vi "LoadNodeUIStandardEvents.vi"(7 "user event out":T1, 8 "error in":errorcluster, 9 "sub panel ref in":refnum<vi>, 10 "main queue":T8, 11 "node":T7) -> (0 "error out":errorcluster)   [LabVIEW 2014, in "NISE_CEF_TreeControl.lvlib"]
doc: "This VI will insert the UI from a node into a subpanel."
uses:
  NISE_CEF_TreeControl.lvlib
  <vilib>/NI/AMC/Message Queue.ctl
  <vilib>/NI/AMC/Message.ctl
  <vilib>/NI/Tools/Keyed Array/KeyedArray.ctl
  Node/NodeRef.ctl
  Node/NISE_CEF_Node.lvclass
  Node/StandardEvents.ctl
  Node/UserEventRef.ctl
  Controls/EventCluster.ctl
  Node/NodeChangeEvent.ctl
  Node/CacheState.ctl
  Node/RefreshUIEvent.ctl
  Node/StopEvent.ctl
  <vilib>/NI/Tools/Keyed Array/Tools_KeyedArray.lvlib
  <vilib>/NI/AMC/AMC.lvlib
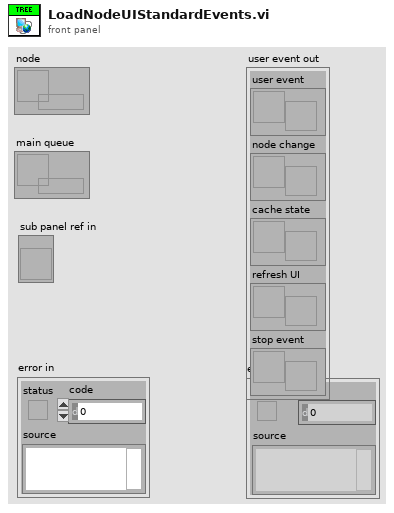
[diagram p1: front panel]
types:
  T1 = typedef "NISE_CEF_Node.lvclass/StandardEvents.ctl" = cluster{"user event":T2, "node change":T3, "cache state":T4, "refresh UI":T5, "stop event":T6}
  T2 = typedef "NISE_CEF_Node.lvclass/UserEventRef.ctl" = refnum<user-event>
  T3 = typedef "NISE_CEF_Node.lvclass/NodeChangeEvent.ctl" = refnum<user-event>
  T4 = typedef "NISE_CEF_Node.lvclass/CacheState.ctl" = refnum<user-event>
  T5 = typedef "NISE_CEF_Node.lvclass/RefreshUIEvent.ctl" = refnum<user-event>
  T6 = typedef "NISE_CEF_Node.lvclass/StopEvent.ctl" = refnum<user-event>
  T7 = typedef "NISE_CEF_Node.lvclass/NodeRef.ctl" = refnum<data-value>
  T8 = typedef "AMC.lvlib/Message Queue.ctl" = refnum<queue>
  T9 = enum32{"Bad", "Idle", "Run top level", "Running"}
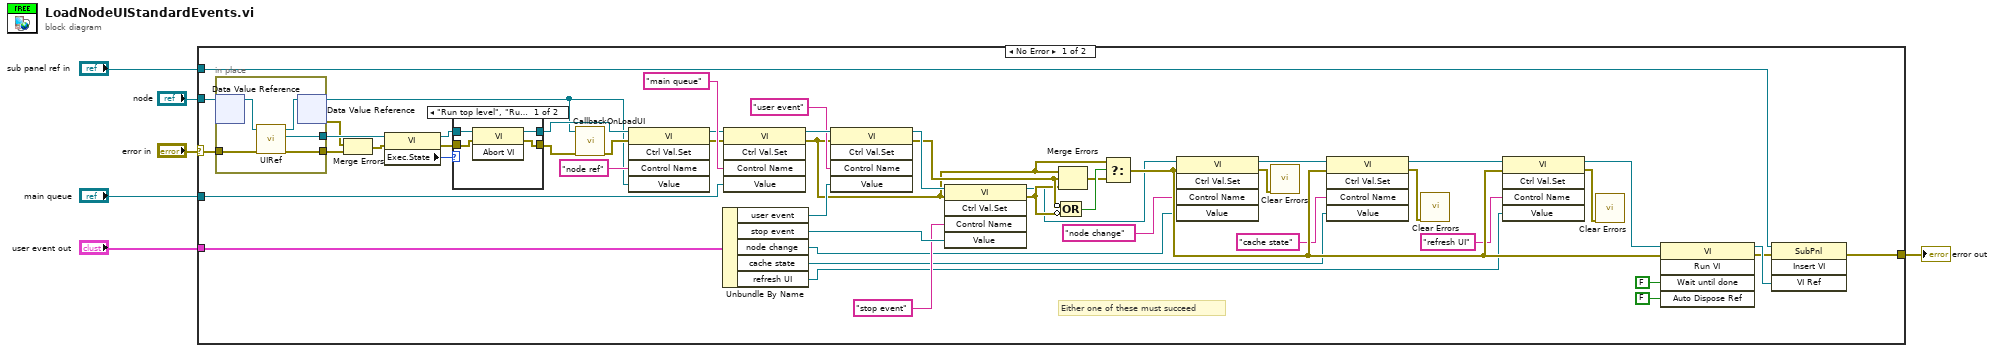
[diagram p0: block diagram]
diagram:
  n1 = case shown="No Error" "error in" {
    selector: "error in" -> [w46 w68]
    tunnel: [w10 w68] -> w5
    tunnel: "node" -> [w40 _]
    tunnel: "main queue" -> [w39 _]
    tunnel: "user event out" -> [w34 _]
    tunnel: "sub panel ref in" -> [w38 _]
    frame No Error {
      # "Either one of these must succeed"
      n2 = in-place {
        in-place-border: w46 -> [w64]
        in-place-border: [w65] -> w45
        in-place-border: [w63] -> w37
        n3 = in-place-dvr #1(w40) -> (w67:refnum<class "NISE_CEF_Node.lvclass">)  [unwired: 1 out]
        n4 = call-dynamic "UIRef.vi"("error in"=w64, "node in"=w67) -> ("error out"=w63:errorcluster, "VI refnum"=w65:refnum<vi>, "node out"=w66:refnum<class "NISE_CEF_Node.lvclass">)  [unwired: 7 in]
        n5 = in-place-dvr #1(w66) -> (w7:T7, w36:errorcluster)
      }
      n6 = Merge Errors(w36, w37) -> (w35:errorcluster)
      n7 = property class="VI"(reference=w45, error in=w35) -> (reference out=w42:refnum<vi>, error out=w41:errorcluster, "Exec.State"=w44:T9)
      n8 = case shown="\"Run top level\", \"Running\"" w44 {
        tunnel: [w57 w62] -> w43
        tunnel: w42 -> [w60 w62]
        tunnel: w41 -> [w59 w61]
        tunnel: [w58 w61] -> w8
        frame "Run top level", "Running" {
          n9 = invoke class="VI" method="Abort VI"(reference=w60, error in=w59) -> (reference out=w57:refnum<vi>, error out=w58:errorcluster)  [unwired: 1 in, 1 out]
        }
        frame "Idle", Default {
        }
      }
      n10 = call "CallbackOnLoadUI.vi"("error in"=w8, "node"=w7) -> ("error out"=w9:errorcluster)  [unwired: 9 in]
      n11 = invoke class="VI" method="Ctrl Val.Set"(reference=w43, error in=w9, "Control Name"="node ref", "Value"=w7) -> (reference out=w54:refnum<vi>, error out=w49:errorcluster)  [unwired: 1 in, 3 out]
      n12 = Unbundle By Name(w34) -> ("user event"=w33:T2, "stop event"=w31:T6, "node change"=w16:T3, "cache state"=w15:T4, "refresh UI"=w14:T5)
      n13 = invoke class="VI" method="Ctrl Val.Set"(reference=w54, error in=w49, "Control Name"="main queue", "Value"=w39) -> (reference out=w48:refnum<vi>, error out=w25:errorcluster)  [unwired: 1 in, 3 out]
      n14 = invoke class="VI" method="Ctrl Val.Set"(reference=w48, error in=w25, "Control Name"="user event", "Value"=w33) -> (reference out=w32:refnum<vi>, error out=w29:errorcluster)  [unwired: 1 in, 3 out]
      n15 = invoke class="VI" method="Ctrl Val.Set"(reference=w32, error in=w25, "Control Name"="stop event", "Value"=w31) -> (reference out=w23:refnum<vi>, error out=w28:errorcluster)  [unwired: 1 in, 3 out]
      n16 = Merge Errors(w25, w29, w28) -> (w26:errorcluster)
      n17 = Compound Arithmetic op=OR(invert w29, invert w28) -> (w27:bool)
      n18 = Select(t=w25, s=w27, f=w26) -> (s? t:f=w24:errorcluster)
      n19 = invoke class="VI" method="Ctrl Val.Set"(reference=w23, error in=w24, "Control Name"="node change", "Value"=w16) -> (reference out=w22:refnum<vi>, error out=w12:errorcluster)  [unwired: 1 in, 3 out]
      n20 = call <vilib>:"Clear Errors.vi"("error in (no error)"=w12) -> ()  [unwired: 5 in, 2 out]
      n21 = invoke class="VI" method="Ctrl Val.Set"(reference=w22, error in=w24, "Control Name"="cache state", "Value"=w15) -> (reference out=w21:refnum<vi>, error out=w13:errorcluster)  [unwired: 1 in, 3 out]
      n22 = call <vilib>:"Clear Errors.vi"("error in (no error)"=w13) -> ()  [unwired: 5 in, 2 out]
      n23 = invoke class="VI" method="Ctrl Val.Set"(reference=w21, error in=w24, "Control Name"="refresh UI", "Value"=w14) -> (reference out=w20:refnum<vi>, error out=w11:errorcluster)  [unwired: 1 in, 3 out]
      n24 = call <vilib>:"Clear Errors.vi"("error in (no error)"=w11) -> ()  [unwired: 5 in, 2 out]
      n25 = invoke class="VI" method="Run VI"(reference=w20, error in=w24, "Wait until done"=FALSE ("Wait Until Done"), "Auto Dispose Ref"=FALSE ("Auto Dispose Reference")) -> (reference out=w53:refnum<vi>, error out=w52:errorcluster)  [unwired: 1 in, 3 out]
      n26 = invoke class="SubPnl" method="Insert VI"(reference=w38, error in=w52, "VI Ref"=w53) -> (error out=w10:errorcluster)  [unwired: 1 in, 3 out]
    }
    frame Error {
    }
  }
  "error out" <- w5
